vi "GetLatestTimes.vi"(8 "error in (no error)":errorcluster, 11 "FAMM in":refnum<class "FAMM.lvclass">) -> (0 "error out":errorcluster, 1 "AverTimes":timestamp[](array[timestamp]), 2 "LatestTimes":timestamp[](array[timestamp]), 3 "FAMM out":refnum<class "FAMM.lvclass">)   [LabVIEW 2020]
doc: "Get the latest times from all the PAQ resolution layers the FAMM buffer"
uses:
  FAMM.lvclass
  DBAL/DBAL.lvclass
  PAQ-memory.lvclass
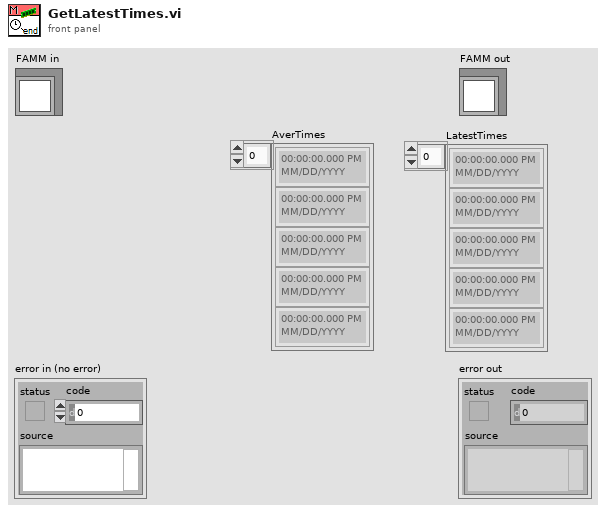
[diagram p1: front panel]
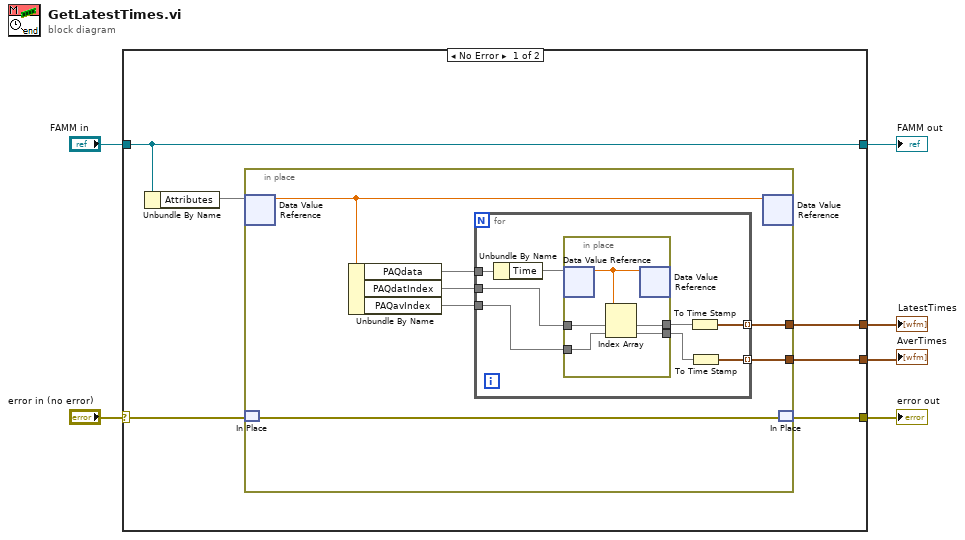
[diagram p0: block diagram]
diagram:
  n1 = case shown="No Error" "error in (no error)" {
    selector: "error in (no error)" -> [w12 w34]
    tunnel: [w11 w34] -> w5
    tunnel: [w8 w33] -> w3
    tunnel: "FAMM in" -> [w8 w33]
    tunnel: [w10 _] -> w2
    tunnel: [w9 _] -> w1
    frame No Error {
      n2 = Unbundle By Name(w8) -> ("Attributes"=w7)
      n3 = in-place {
        in-place-border: [w17] -> w10
        in-place-border: [w13] -> w9
        n4 = in-place-dvr #1(w7) -> (w19:dbl)  [unwired: 1 out]
        n5 = in-place-match #2(w12) -> (w18:errorcluster)
        n6 = Unbundle By Name(w19) -> ("PAQdata"=w16, "PAQdatIndex"=w15, "PAQavIndex"=w14)
        n7 = for {
          tunnel: w16 -> [w27]
          tunnel: w15 -> [w25]
          tunnel: [w23] -> w17 mode=indexing
          tunnel: w14 -> [w22]
          tunnel: [w20] -> w13 mode=indexing
          n8 = Unbundle By Name(w27) -> ("Time"=w26)
          n9 = in-place {
            in-place-border: w25 -> [w31]
            in-place-border: [w30] -> w24
            in-place-border: w22 -> [w29]
            in-place-border: [w28] -> w21
            n10 = in-place-dvr #3(w26) -> (w32:dbl)  [unwired: 1 out]
            n11 = Index Array(array=w32, index #1=w31, index #2=w29) -> (element #1=w30, element #2=w28)
            n12 = in-place-dvr #3(w32) -> ()  [unwired: 2 out]
          }
          n13 = To Time Stamp(1:w24) -> (0:w23:timestamp)
          n14 = To Time Stamp(1:w21) -> (0:w20:timestamp)
        }
        n15 = in-place-dvr #1(w19) -> ()  [unwired: 2 out]
        n16 = in-place-match #2(w18) -> (w11:errorcluster)
      }
    }
    frame Error {
    }
  }
  "error out" <- w5
  "FAMM out" <- w3
  "LatestTimes" <- w2
  "AverTimes" <- w1
